vi "String to Build Version.vi"(8 "error in":errorcluster, 11 "Version String":string) -> (0 "error out":errorcluster, 3 "Build Specification Version":T1)   [LabVIEW 2026]
doc: "This VI tranforms a string version into a build specification version object."
uses:
  <vilib>/AppBuilder/AB_API_Simple/Build Specification Version.ctl
  <vilib>/regexp/Match Regular Expression.xnode
  <vilib>/AppBuilder/AB_API_Simple/NI_App_Builder_API.lvlib
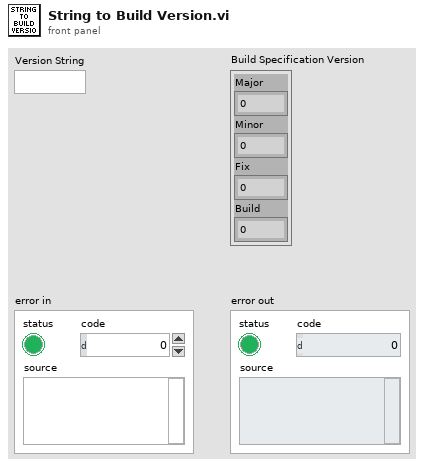
[diagram p1: front panel]
types:
  T1 = typedef "NI_App_Builder_API.lvlib/Build Specification Version.ctl" = cluster{"Major":u16, "Minor":u16, "Fix":u16, "Build":u16}
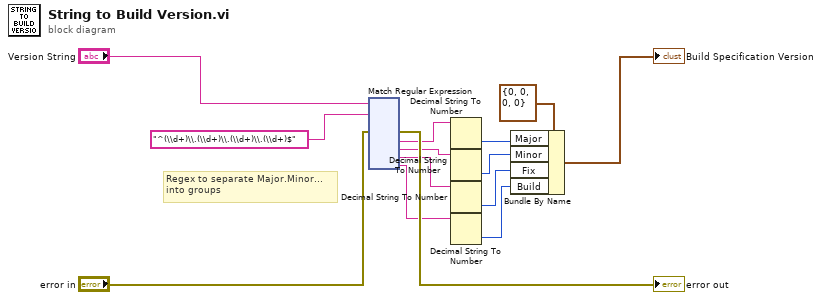
[diagram p0: block diagram]
diagram:
  # "Regex to separate Major.Minor...\ninto groups"
  n1 = xnode "Match Regular Expression"("input string"="Version String", "regular expression"="^(\\d+)\\.(\\d+)\\.(\\d+)\\.(\\d+)$", "error in"="error in") -> ("error out"=→"error out":errorcluster, "submatch 1"=w10:string, "submatch 2"=w9:string, "submatch 3"=w8:string, "submatch 4"=w7:string)  [unwired: 3 in, 4 out]
  n2 = Decimal String To Number(string=w10) -> (number=w3:i32)  [unwired: 2 in, 1 out]
  n3 = Decimal String To Number(string=w9) -> (number=w4:i32)  [unwired: 2 in, 1 out]
  n4 = Decimal String To Number(string=w8) -> (number=w5:i32)  [unwired: 2 in, 1 out]
  n5 = Decimal String To Number(string=w7) -> (number=w6:i32)  [unwired: 2 in, 1 out]
  n6 = Bundle By Name(cluster=T1 {"Major"=0, "Minor"=0, "Fix"=0, "Build"=0} ("Build Specification Version"), "Major"=w3, "Minor"=w4, "Fix"=w5, "Build"=w6) -> (→"Build Specification Version":T1)
